vi "RP1210 Read Message.vi"(8 "error in (no error)":errorcluster, 9 "nBlockOnRead":i16, 10 "nBufferSize":i16=64, 11 "nClientID":i16) -> (0 "error out":errorcluster, 2 "function return":i16, 3 "fpchAPIMessage":u8[](array[numeric]))   [LabVIEW 2020, in "cansub_rp1210.lvlib"]
doc: "short __stdcall RP1210_ReadMessage(short nClientID, unsigned char fpchAPIMessage[], short nBufferSize,\n short nBlockOnRead);"
uses:
  cansub_rp1210.lvlib
  cansub_lv64.dll
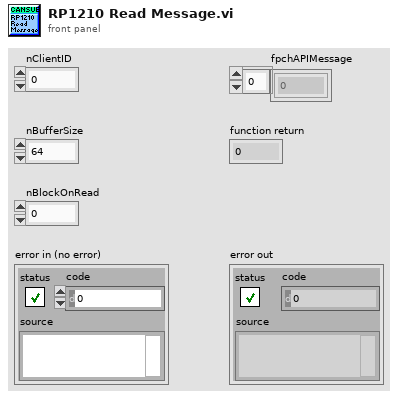
[diagram p1: front panel]
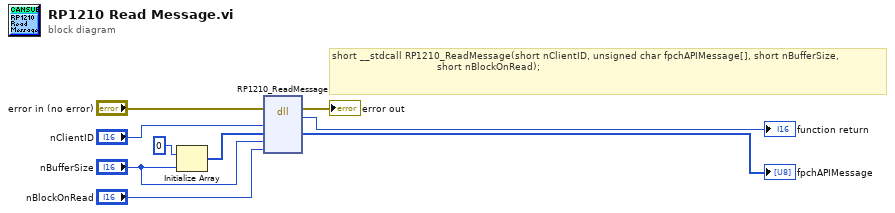
[diagram p0: block diagram]
diagram:
  # "short __stdcall RP1210_ReadMessage(short nClientID, unsigned char fpchAPIMessage[], short nBufferSize,\n                                   short nBlockOnRead);"
  n1 = Initialize Array(u8 0 ("element"), "nBufferSize") -> (w7:u8[])
  n2 = dll-call lib="C:/cansub-lv/library/cansub_lv*.*" fn="RP1210_ReadMessage"(error in="error in (no error)", "nClientID"="nClientID", "fpchAPIMessage"=w7, "nBufferSize"="nBufferSize", "nBlockOnRead"="nBlockOnRead") -> (error out=→"error out":errorcluster, "return type"=→"function return":i16, "fpchAPIMessage"=→"fpchAPIMessage":u8[])  [unwired: 5 in, 1 out]
